vi "Log Results.vi"(8 "error in (no error)":errorcluster, 11 "Instrument.Lockin in":refnum<class "Instrument.Lockin.lvclass">) -> (0 "error out":errorcluster, 3 "Instrument.Lockin out":refnum<class "Instrument.Lockin.lvclass">)   [LabVIEW 2019, in "Instrument.Lockin.lvlib" / "Instrument.Lockin.lvclass"]
uses:
  Instrument.Lockin.lvclass
  C:/Program Files/National Instruments/LabVIEW 2019/user.lib/LevyLab/Instrument Framework/Instrument/Instrument.lvclass
  Instrument.Lockin.lvclass/Instrument.Lockin.ctl
  Typedefs/Results Type--Enum.ctl
  Typedefs/Lockin.LogSweepXY--Cluster.ctl
  <userlib>/LevyLab/Instrument Framework/Instrument/Instrument.lvclass
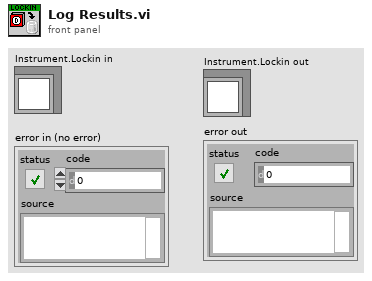
[diagram p1: front panel]
types:
  T1 = typedef "Instrument.Lockin.lvlib/Instrument.Lockin.lvclass/Results Type--Enum.ctl" = enum16{"X", "Y", "R", "Theta", "Mean"}
  T2 = typedef "Instrument.Lockin.lvlib/Instrument.Lockin.lvclass/Lockin.LogSweepXY--Cluster.ctl" = cluster{"SystemSerialNumber":string, "System Channel":i32, "REF Channel":i32, "X":dbl, "Y":dbl, "Sweeping?":bool}
  T3 = typedef "Instrument.Lockin.lvlib/Instrument.DAQ.lvclass/DeviceInfo--Cluster.ctl" = cluster{"DeviceName":string, "DevIsSimulated":bool, "DeviceSerialNumber":string, "ProductType":string, "ProductCategory":i32, "ProductNumber":u32, "ChassisNumber":u32, "SlotNumber":u32, "ChassisName":string, "ChassisSerialNumber":string, "DevTemp":dbl, "SelfCal.LastDate/Time":string, "SelfCal.LastTemp":dbl, "calibration due?":bool}
  T4 = typedef "Instrument.Lockin.lvlib/Instrument.DAQ.lvclass/Results--Cluster.ctl" = cluster{"Time Stamp":timestamp, "Results (Dictionary)":cluster{"key":string, "value":dbl[]}[]}
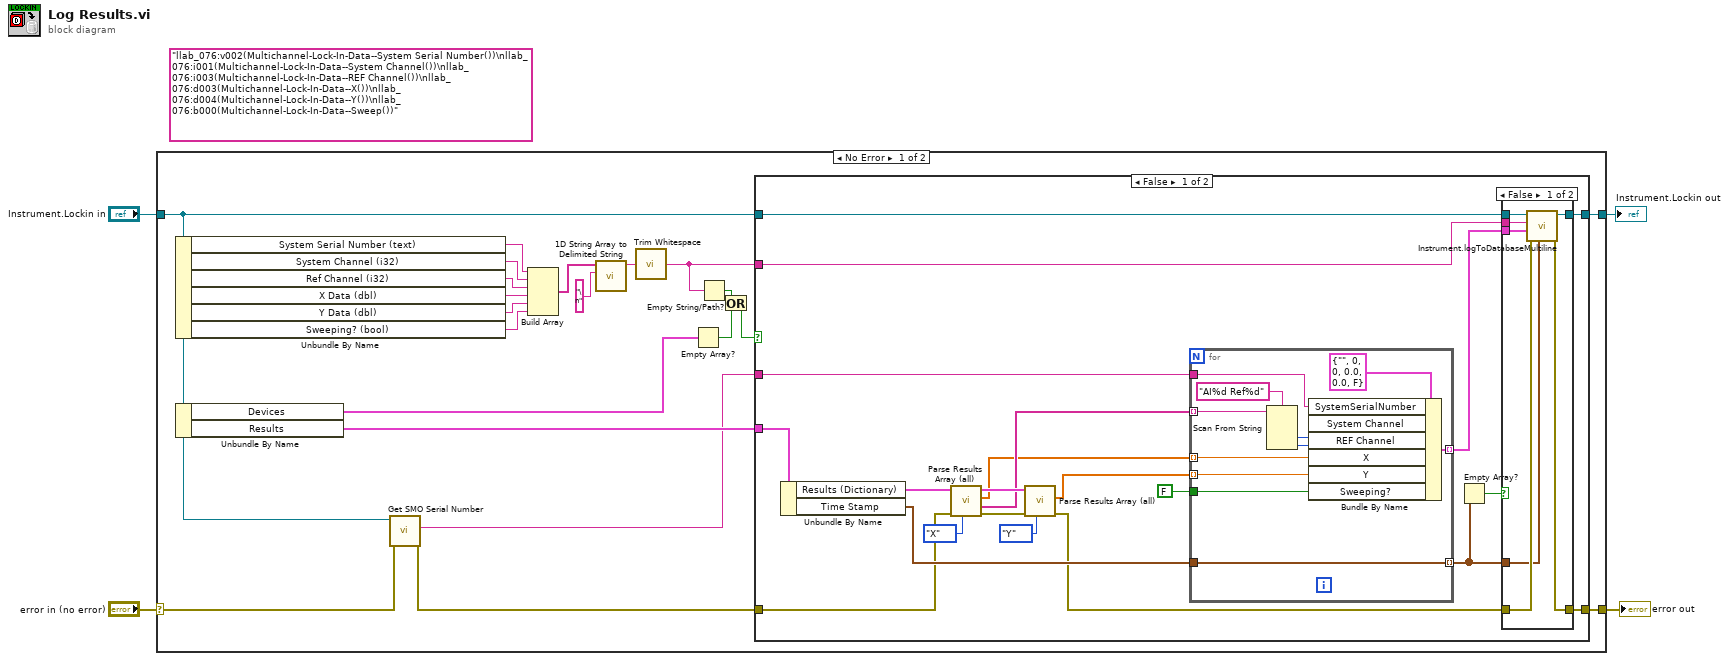
[diagram p0: block diagram]
diagram:
  (unwired) "llab_076:v002(Multichannel-Lock-In-Data--System Serial Number())\nllab_076:i001(Multichannel-Lock-In-Data--System Channel())\nllab_076:i003(Multichannel-Lock-In-Data--REF Channel())\nllab_076:d003(Multichannel-Lock-In-Data--X())\nllab_076:d004(Multichannel-Lock-In-Data--Y())\nllab_076:b000(Multichannel-Lock-In-Data--Sweep())"
  n1 = case shown="No Error" "error in (no error)" {
    selector: "error in (no error)" -> [w9 w70]
    tunnel: "Instrument.Lockin in" -> [w10 w69]
    tunnel: [w25 w70] -> w3
    tunnel: [w13 w69] -> w1
    frame No Error {
      n2 = Unbundle By Name(w10) -> ("System Serial Number (text)"=w18:string, "System Channel (i32)"=w23:string, "Ref Channel (i32)"=w22:string, "X Data (dbl)"=w21:string, "Y Data (dbl)"=w20:string, "Sweeping? (bool)"=w19:string)
      n3 = Unbundle By Name(w10) -> ("Devices"=w6:T3[], "Results"=w24:T4)
      n4 = call-dynamic "Get SMO Serial Number.vi"("error in (no error)"=w9, "Instrument.Lockin in"=w10) -> ("error out"=w8:errorcluster, "Serial Number"=w7:string)  [unwired: 7 in, 1 out]
      n5 = Build Array(w18, w23, w22, w21, w20, w19) -> (w5:string[])
      n6 = call <vilib>:"1D String Array to Delimited String.vi"("delimiter"="\n", "string array"=w5) -> ("delimited string"=w12:string)  [unwired: 9 in]
      n7 = call <vilib>:"Trim Whitespace.vi"("string"=w12) -> ("trimmed string"=w11:string)  [unwired: 1 in]
      n8 = Empty Array?(array=w6) -> (empty?=w16:bool)
      n9 = Empty String/Path?(string/path=w11) -> (empty?=w14:bool)
      n10 = Or(x=w14, y=w16) -> (x .or. y?=w15:bool)
      n11 = case shown="False" w15 {
        tunnel: w10 -> [w46 w67]
        tunnel: [w45 w68] -> w25
        tunnel: w8 -> [w34 w68]
        tunnel: w24 -> [w28 _]
        tunnel: w11 -> [w31 _]
        tunnel: [w30 w67] -> w13
        tunnel: w7 -> [w29 _]
        frame False {
          n12 = Unbundle By Name(w28) -> ("Results (Dictionary)"=w44:cluster{"key":string, "value":dbl[]}[], "Time Stamp"=w36:timestamp)
          n13 = call "Parse Results Array (all).vi"("Type"=Results_Type--Enum."X", "error in (no error)"=w34, "Results (Dictionary)"=w44) -> ("error out"=w40:errorcluster, "Label"=w39:string[], "Data"=w27:dbl[], "Results (Dictionary)"=w41:cluster{"key":string, "value":dbl[]}[])  [unwired: 5 in]
          n14 = call "Parse Results Array (all).vi"("Type"=Results_Type--Enum."Y", "error in (no error)"=w40, "Results (Dictionary)"=w41) -> ("error out"=w35:errorcluster, "Data"=w26:dbl[])  [unwired: 5 in, 2 out]
          n15 = for {
            tunnel: w29 -> [w57]
            tunnel: w27 -> [w47] mode=indexing
            tunnel: w26 -> [w56] mode=indexing
            tunnel: w39 -> [w52] mode=indexing
            tunnel: [w51] -> w33 mode=indexing
            tunnel: w36 -> [w50]
            tunnel: [w50] -> w37 mode=indexing
            tunnel: FALSE -> [w49]
            n16 = Scan From String(format string="AI%d Ref%d", input string=w52) -> (output 1=w54:i32, output 2=w53:i32)  [unwired: 4 in, 3 out]
            n17 = Bundle By Name(cluster=T2 {"SystemSerialNumber"="", "System Channel"=0, "REF Channel"=0, "X"=0.0, "Y"=0.0, "Sweeping?"=FALSE}, "SystemSerialNumber"=w57, "System Channel"=w54, "REF Channel"=w53, "X"=w47, "Y"=w56, "Sweeping?"=w49) -> (w51:T2)
          }
          n18 = Empty Array?(array=w37) -> (empty?=w32:bool)
          n19 = case shown="False" w32 {
            tunnel: w46 -> [w64 w65]
            tunnel: [w63 w66] -> w45
            tunnel: w35 -> [w62 w66]
            tunnel: w31 -> [w61 _]
            tunnel: w33 -> [w60 _]
            tunnel: w37 -> [w59 _]
            tunnel: [w58 w65] -> w30
            frame False {
              n20 = call <userlib>:"Instrument.logToDatabaseMultiline.vi"("timestamps"=w59, "error in (no error)"=w62, "Data"=w60, "Paths"=w61, "Instrument"=w64) -> ("error out"=w63:errorcluster, "Instrument out"=w58:refnum<class "Instrument.Lockin.lvclass">)  [unwired: 5 in]
            }
            frame True {
            }
          }
        }
        frame True {
        }
      }
    }
    frame Error {
    }
  }
  "error out" <- w3
  "Instrument.Lockin out" <- w1
